vi "JSON Tree Base Type to String.vi"(8 "error in (no error)":errorcluster, 11 "JSON Tree Base Type":variant) -> (0 "error out":errorcluster, 2 "JSON Tree Base Type String":string)   [LabVIEW 2014, in "i3-json.lvlib"]
doc: "Flattens a node's base type to a string"
uses:
  i3-json.lvlib
  JSON Types/JSON Type.ctl
  JSON Types/JSON Variant Attribute.ctl
  JSON Types/JSON Compatible Type.ctl
  Generation Error.ctl
  JSON Types/JSON Value String.ctl
  Error Handling/Throw JSON Error Files/Throw JSON Error - Creation Error.vi
  Error Handling/Throw JSON Error Files/Throw JSON Error - Invalid Type Error.vi
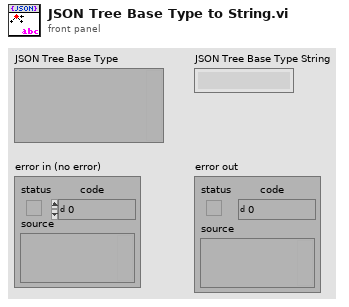
[diagram p1: front panel]
types:
  T1 = typedef "i3-json.lvlib/JSON Type.ctl" = enum8{"JSON Compatible", "JSON Array", "JSON Object", "JSON Null", "Double", "String", "Boolean", "Unknown"}
  T2 = typedef "i3-json.lvlib/JSON Variant Attribute.ctl" = string
  T3 = typedef "i3-json.lvlib/JSON Compatible Type.ctl" = enum16{"1D Double Array", "1D String Array", "1D Boolean Array", "Unknown"}
  T4 = typedef "i3-json.lvlib/Generation Error.ctl" = string
  T5 = typedef "i3-json.lvlib/JSON Value String.ctl" = string
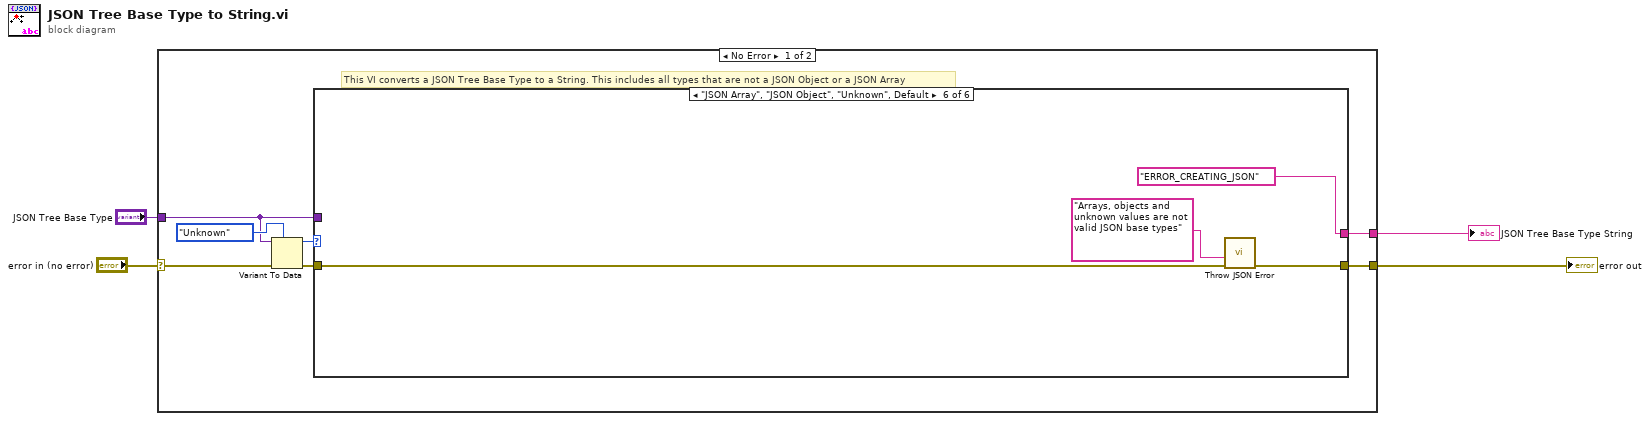
[diagram p0: block diagram]
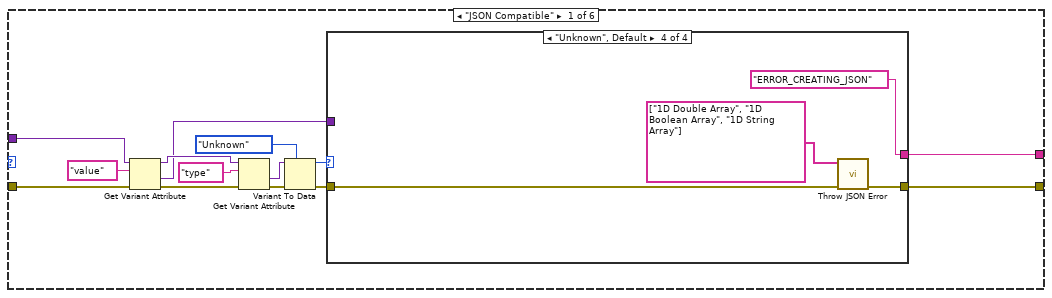
[diagram p2: hidden frame]
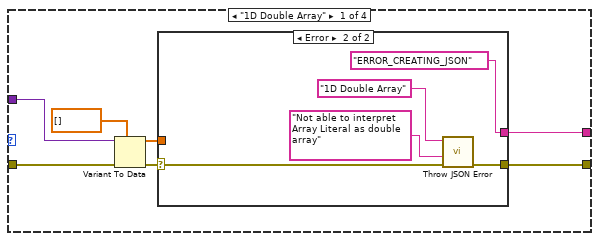
[diagram p3: hidden frame]
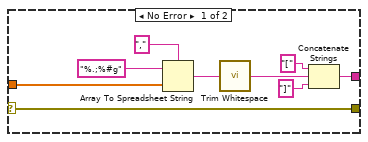
[diagram p4: hidden frame]
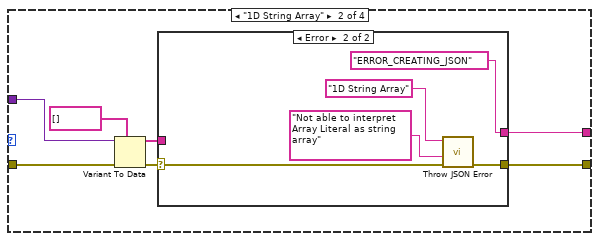
[diagram p5: hidden frame]
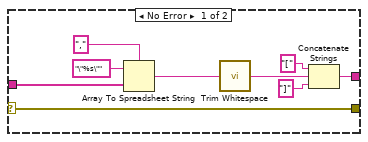
[diagram p6: hidden frame]
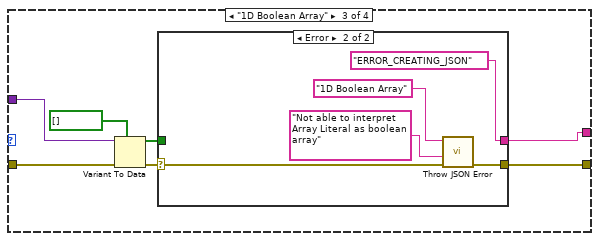
[diagram p7: hidden frame]
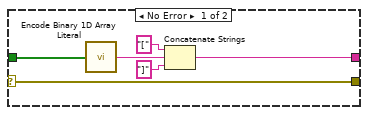
[diagram p8: hidden frame]
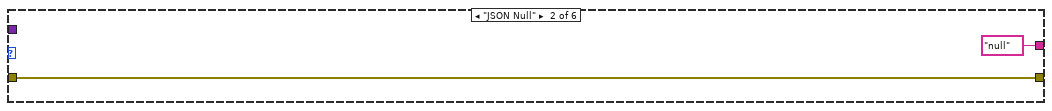
[diagram p9: hidden frame]
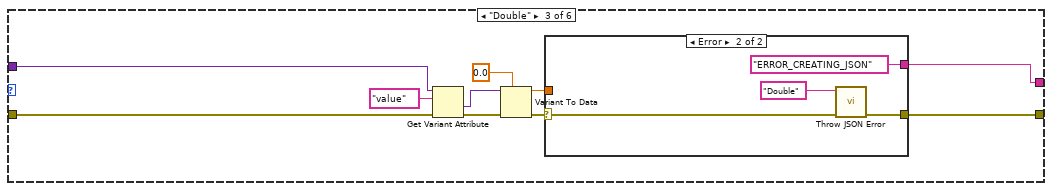
[diagram p10: hidden frame]
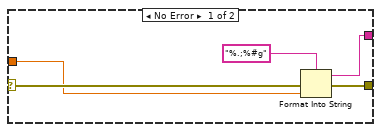
[diagram p11: hidden frame]
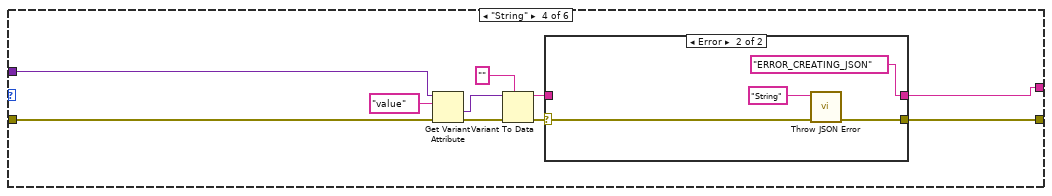
[diagram p12: hidden frame]
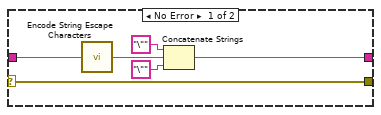
[diagram p13: hidden frame]
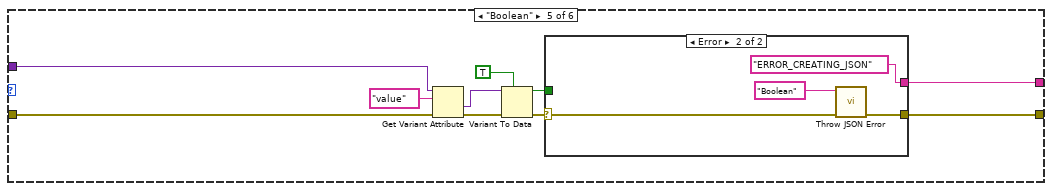
[diagram p14: hidden frame]
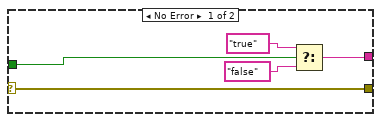
[diagram p15: hidden frame]
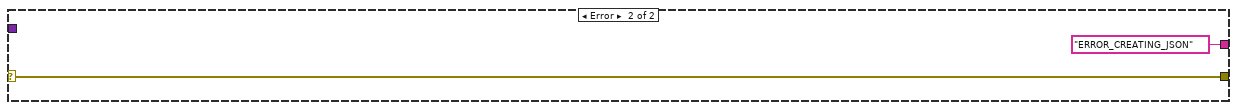
[diagram p16: hidden frame]
diagram:
  n1 = case shown="No Error" "error in (no error)" {
    selector: "error in (no error)" -> [w11 w155]
    tunnel: [w8 w155] -> w3
    tunnel: [w6 T4 "ERROR_CREATING_JSON" ("Generating Error")] -> w2
    tunnel: "JSON Tree Base Type" -> [w5 _]
    frame No Error {
      # "This VI converts a JSON Tree Base Type to a String. This includes all types that are not a JSON Object or a JSON Array"
      n2 = Variant To Data(error in=w11, type=JSON_Type."Unknown" ("JSON Type"), Variant=w5) -> (data=w9:T1, error out=w7:errorcluster)
      n3 = case shown="\"JSON Array\", \"JSON Object\", \"Unknown\", Default" w9 {
        tunnel: [w15 T5 "null" ("JSON Value String") w97 w113 w133 T4 "ERROR_CREATING_JSON" ("Generating Error")] -> w6
        tunnel: [w14 w90 w98 w114 w134 w150] -> w8
        tunnel: w7 -> [w13 w90 w92 w111 w131 w151]
        tunnel: w5 -> [w12 _ w96 w112 w132 _]
        frame "JSON Compatible" {
          n4 = Get Variant Attribute(Variant=w12, name=T2 "value" ("JSON Variant Attribute"), error in=w13) -> (duplicate Variant=w19:variant, value=w16:variant, error out=w18:errorcluster)  [unwired: 1 in, 1 out]
          n5 = Get Variant Attribute(Variant=w19, name=T2 "type" ("JSON Variant Attribute"), error in=w18) -> (value=w24:variant, error out=w22:errorcluster)  [unwired: 1 in, 2 out]
          n6 = Variant To Data(error in=w22, type=JSON_Compatible_Type."Unknown" ("JSON Compatible Type"), Variant=w24) -> (data=w21:T3, error out=w20:errorcluster)
          n7 = case shown="\"Unknown\", Default" w21 {
            tunnel: w20 -> [w31 w49 w72 w88]
            tunnel: [w28 w47 w69 w87] -> w14
            tunnel: w16 -> [w32 w50 w71 _]
            tunnel: [w26 w48 w68 T4 "ERROR_CREATING_JSON" ("Generating Error")] -> w15
            frame "1D Double Array" {
              n8 = Variant To Data(error in=w31, type=dbl[] [], Variant=w32) -> (data=w27:dbl[], error out=w29:errorcluster)
              n9 = case shown="Error" w29 {
                selector: w29 -> [w34 w43]
                tunnel: [w34 w42] -> w28
                tunnel: w27 -> [w41 _]
                tunnel: [w35 T4 "ERROR_CREATING_JSON" ("Generating Error")] -> w26
                frame No Error {
                  n10 = Array To Spreadsheet String(delimiter (Tab)=",", array=w41, 3:"%.;%#g" ("format string")) -> (spreadsheet string=w37:string)
                  n11 = call <vilib>:"Trim Whitespace.vi"("string"=w37) -> ("trimmed string"=w33:string)  [unwired: 1 in]
                  n12 = Concatenate Strings("[" ("string"), w33, "]" ("string")) -> (w35:string)
                }
                frame Error {
                  n13 = call-poly "Throw JSON Error.vi"("error in (no error)"=w43, "additional info"="Not able to interpret Array Literal as double array" ("source"), "datatype"="1D Double Array") -> ("error out"=w42:errorcluster)  [unwired: 8 in]
                }
              }
            }
            frame "1D String Array" {
              n14 = Variant To Data(error in=w49, type=string[] [], Variant=w50) -> (data=w51:string[], error out=w52:errorcluster)
              n15 = case shown="Error" w52 {
                selector: w52 -> [w55 w64]
                tunnel: [w55 w63] -> w47
                tunnel: w51 -> [w62 _]
                tunnel: [w56 T4 "ERROR_CREATING_JSON" ("Generating Error")] -> w48
                frame No Error {
                  n16 = Array To Spreadsheet String(delimiter (Tab)=",", array=w62, 3:"\"%s\"" ("format string")) -> (spreadsheet string=w58:string)
                  n17 = call <vilib>:"Trim Whitespace.vi"("string"=w58) -> ("trimmed string"=w54:string)  [unwired: 1 in]
                  n18 = Concatenate Strings("[" ("string"), w54, "]" ("string")) -> (w56:string)
                }
                frame Error {
                  n19 = call-poly "Throw JSON Error.vi"("error in (no error)"=w64, "additional info"="Not able to interpret Array Literal as string array" ("source"), "datatype"="1D String Array") -> ("error out"=w63:errorcluster)  [unwired: 8 in]
                }
              }
            }
            frame "1D Boolean Array" {
              n20 = Variant To Data(error in=w72, type=bool[] [], Variant=w71) -> (data=w73:bool[], error out=w70:errorcluster)
              n21 = case shown="Error" w70 {
                selector: w70 -> [w77 w82]
                tunnel: [w77 w81] -> w69
                tunnel: w73 -> [w75 _]
                tunnel: [w78 T4 "ERROR_CREATING_JSON" ("Generating Error")] -> w68
                frame No Error {
                  n22 = call "Encode Binary 1D Array Literal.vi"("Array"=w75) -> ("string"=w76:string)
                  n23 = Concatenate Strings("[" ("string"), w76, "]" ("string")) -> (w78:string)
                }
                frame Error {
                  n24 = call-poly "Throw JSON Error.vi"("error in (no error)"=w82, "additional info"="Not able to interpret Array Literal as boolean array" ("source"), "datatype"="1D Boolean Array") -> ("error out"=w81:errorcluster)  [unwired: 8 in]
                }
              }
            }
            frame "Unknown", Default {
              n25 = call-poly "Throw JSON Error.vi"("error in (no error)"=w88, "Valid Types"=string[] ["1D Double Array", "1D Boolean Array", "1D String Array"]) -> ("error out"=w87:errorcluster)  [unwired: 9 in]
            }
          }
        }
        frame "JSON Null" {
        }
        frame "Double" {
          n26 = Get Variant Attribute(Variant=w96, name=T2 "value" ("JSON Variant Attribute"), error in=w92) -> (value=w95:variant, error out=w94:errorcluster)  [unwired: 1 in, 2 out]
          n27 = Variant To Data(error in=w94, type=0.0, Variant=w95) -> (data=w99:dbl, error out=w100:errorcluster)
          n28 = case shown="Error" w100 {
            selector: w100 -> [w106 w109]
            tunnel: w99 -> [w105 _]
            tunnel: [w102 w108] -> w98
            tunnel: [w103 T4 "ERROR_CREATING_JSON" ("Generating Error")] -> w97
            frame No Error {
              n29 = Format Into String(format string="%.;%#g", error in=w106, w105) -> (resulting string=w103:string, error out=w102:errorcluster)  [unwired: 1 in]
            }
            frame Error {
              n30 = call-poly "Throw JSON Error.vi"("error in (no error)"=w109, "datatype"="Double") -> ("error out"=w108:errorcluster)  [unwired: 9 in]
            }
          }
        }
        frame "String" {
          n31 = Get Variant Attribute(Variant=w112, name=T2 "value" ("JSON Variant Attribute"), error in=w111) -> (value=w118:variant, error out=w116:errorcluster)  [unwired: 1 in, 2 out]
          n32 = Variant To Data(error in=w116, type="", Variant=w118) -> (data=w120:string, error out=w119:errorcluster)
          n33 = case shown="Error" w119 {
            selector: w119 -> [w126 w128]
            tunnel: w120 -> [w122 _]
            tunnel: [w126 w127] -> w114
            tunnel: [w125 T4 "ERROR_CREATING_JSON" ("Generating Error")] -> w113
            frame No Error {
              n34 = call "Encode String Escape Characters.vi"("unescaped string in"=w122) -> ("escaped string out"=w121:string)
              n35 = Concatenate Strings("\"" ("string"), w121, "\"" ("string")) -> (w125:string)
            }
            frame Error {
              n36 = call-poly "Throw JSON Error.vi"("error in (no error)"=w128, "datatype"="String") -> ("error out"=w127:errorcluster)  [unwired: 9 in]
            }
          }
        }
        frame "Boolean" {
          n37 = Get Variant Attribute(Variant=w132, name=T2 "value" ("JSON Variant Attribute"), error in=w131) -> (value=w138:variant, error out=w137:errorcluster)  [unwired: 1 in, 2 out]
          n38 = Variant To Data(error in=w137, type=TRUE, Variant=w138) -> (data=w140:bool, error out=w139:errorcluster)
          n39 = case shown="Error" w139 {
            selector: w139 -> [w145 w147]
            tunnel: w140 -> [w144 _]
            tunnel: [w145 w146] -> w134
            tunnel: [w141 T4 "ERROR_CREATING_JSON" ("Generating Error")] -> w133
            frame No Error {
              n40 = Select(t=T5 "true" ("JSON Value String"), s=w144, f=T5 "false" ("JSON Value String")) -> (s? t:f=w141:T5)
            }
            frame Error {
              n41 = call-poly "Throw JSON Error.vi"("error in (no error)"=w147, "datatype"="Boolean") -> ("error out"=w146:errorcluster)  [unwired: 9 in]
            }
          }
        }
        frame "JSON Array", "JSON Object", "Unknown", Default {
          n42 = call-poly "Throw JSON Error.vi"("error in (no error)"=w151, "additional info"="Arrays, objects and unknown values are not valid JSON base types" ("source")) -> ("error out"=w150:errorcluster)  [unwired: 9 in]
        }
      }
    }
    frame Error {
    }
  }
  "error out" <- w3
  "JSON Tree Base Type String" <- w2
